vi "Check failure.vi"(8 "error in":errorcluster, 11 "VISA resource name":refnum<visa-resource-name>) -> (0 "error out":errorcluster, 2 "Result":bool, 3 "VISA resource name out":refnum<visa-resource-name>)   [LabVIEW 2021]
uses:
  GPT-9800_GSB_L8.5/GPT-9000.lvlib
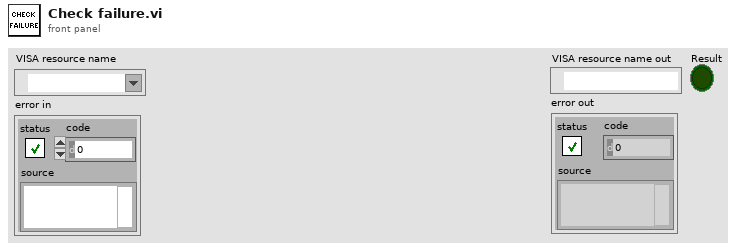
[diagram p1: front panel]
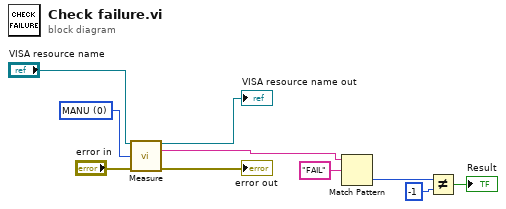
[diagram p0: block diagram]
diagram:
  w9 = u8 0 items=["MANU", "AUTO"] ("Function Mode Numeric")
  n1 = call "Measure.vi"("VISA resource name"="VISA resource name", "Function Mode Numeric"=w9, "error in"="error in") -> ("VISA resource name out"=→"VISA resource name out":refnum<visa-resource-name>, "Return  the test status"=w1:string, "error out"=→"error out":errorcluster)  [unwired: 9 in, 1 out]
  n2 = Match Pattern(string=w1, regular expression="FAIL") -> (offset past match=w4:i32)  [unwired: 1 in, 3 out]
  n3 = Not Equal?(x=w4, y=-1) -> (x != y?=→"Result":bool)
